vi "imaging_echoes__2743b9f66e.vi"(6 "offset (sec)":dbl=0.005, 7 "trigger voltage":dbl=3.8 format="%0.2f", 9 "frames/period":dbl=10.0, 10 "Exposure (s)":dbl=0.0001, 11 "frequency":dbl) -> (3 "output array":cluster{dbl, dbl}[](array[cluster]))   [LabVIEW 2023]
uses:
  <vilib>/Utility/error.llb/DialogType.ctl
  <vilib>/DAQmx/write.llb/DAQmx Write (Analog DBL 1Chan 1Samp).vi
  <vilib>/DAQmx/write.llb/DAQmx Write (Counter 1D Time 1Chan NSamp).vi
  <vilib>/DAQmx/create/channels.llb/DAQmx Create Channel (AO-Voltage-Basic).vi
  <vilib>/DAQmx/miscellaneous.llb/DAQmx Fill In Error Info.vi
  <vilib>/DAQmx/create/channels.llb/DAQmx Create Channel (CO-Pulse Generation-Time).vi
  <vilib>/DAQmx/configure/trigger.llb/DAQmx Start Trigger (Digital Edge).vi
  <vilib>/DAQmx/configure/timing.llb/DAQmx Timing (Implicit).vi
  <resource>/objmgr/daqmx.rc
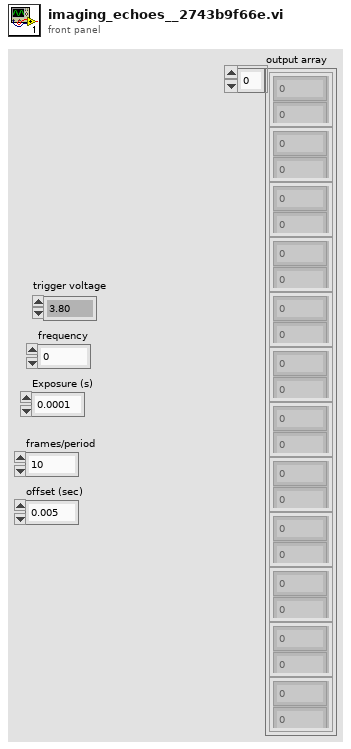
[diagram p1: front panel]
types:
  T1 = typedef "DialogType.ctl" = u16
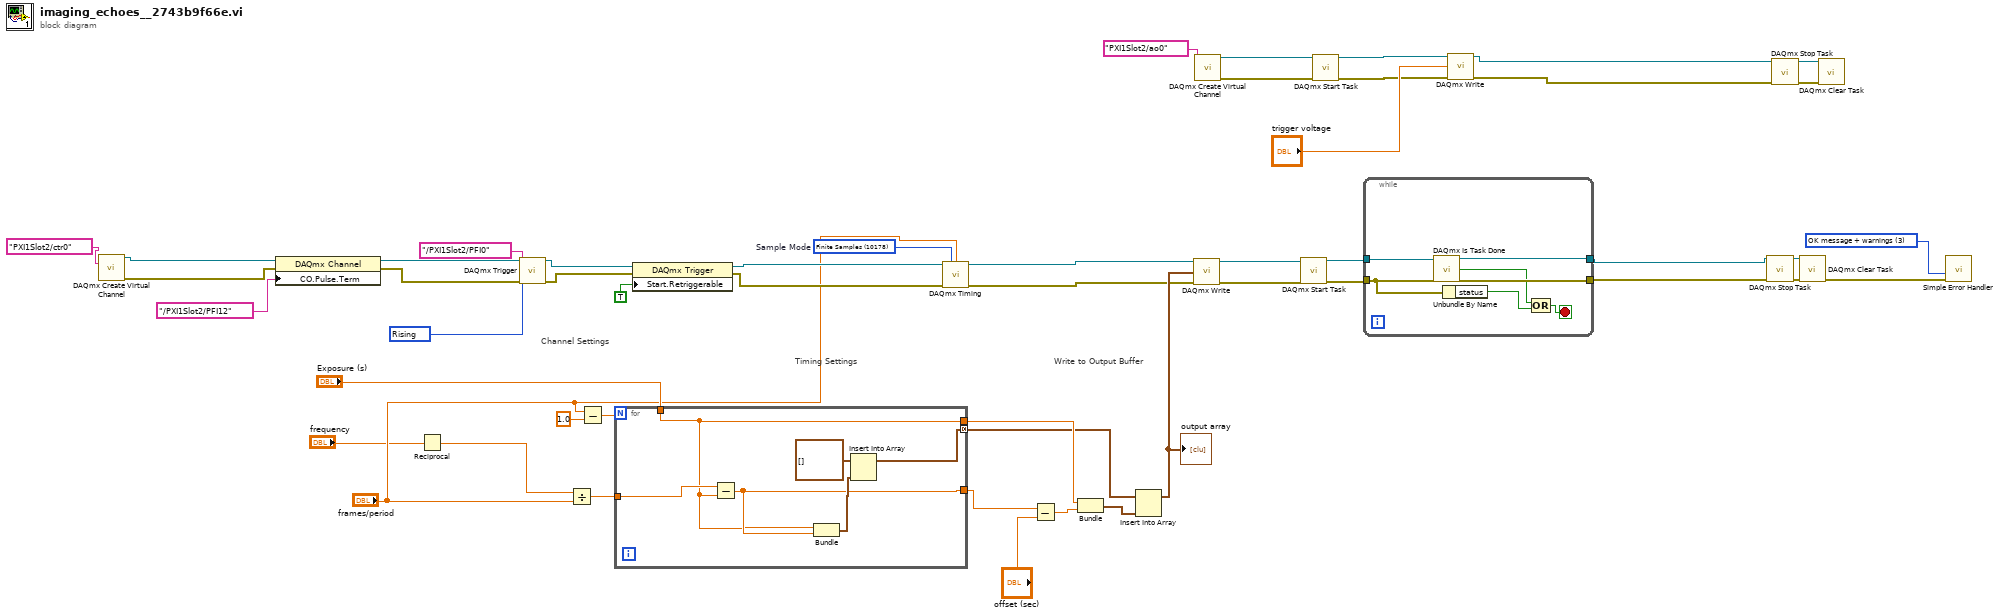
[diagram p0: block diagram]
diagram:
  w47 = 10178 items=["Finite Samples"=10178, "Continuous Samples"=10123, "Hardware Timed Single Point"=12522]  # Sample Mode
  w15 = 10280 items=["Rising"=10280, "Falling"=10171] ("edge")
  w11 = T1 3 items=["no dialog", "OK message", "continue or stop message", "OK message + warnings", "continue/stop + warnings"] ("type of dialog (OK msg:1)")
  # "Write to Output Buffer"
  # "Timing Settings"
  # "Channel Settings"
  n1 = call-poly <vilib>:"DAQmx Create Virtual Channel.vi"("counter"=tag "PXI1Slot2/ctr0") -> ("task out"=w49:refnum<k21>, "error out"=w50:errorcluster)  [unwired: 13 in]
  n2 = property class="DAQmx Channel"(reference=w49, error in=w50, "CO.Pulse.Term"=tag "/PXI1Slot2/PFI12") -> (reference out=w12:refnum<k21>, error out=w13:errorcluster)
  n3 = Reciprocal(x="frequency") -> (1/x=w44:dbl)
  n4 = call-poly <vilib>:"DAQmx Trigger.vi"("task/channels in"=w12, "source"=tag "/PXI1Slot2/PFI0", "edge"=w15, "error in"=w13) -> ("task out"=w16:refnum<k21>, "error out"=w17:errorcluster)  [unwired: 10 in]
  n5 = Divide(x=w44, y="frames/period") -> (x/y=w19:dbl)
  n6 = Subtract(x="frames/period", y=1.0) -> (x-y=w20:dbl)
  n7 = for {
    N: w20 -> [_]
    tunnel: [w54] -> w24 mode=concatenating
    tunnel: w19 -> [w56]
    tunnel: [w52] -> w22
    tunnel: [w51] -> w25
    tunnel: "Exposure (s)" -> [w51]
    n8 = Subtract(x=w56, y=w51) -> (x-y=w52:dbl)
    n9 = Bundle("Exposure (s)"=w51, w52) -> (w55:cluster{"Exposure (s)":dbl, dbl})  [unwired: 1 in]
    n10 = Insert Into Array(array=cluster{dbl, dbl}[] [], new element=w55) -> (w54:cluster{dbl, dbl}[])  [unwired: 1 in]
  }
  n11 = property class="DAQmx Trigger"(reference=w16, error in=w17, "Start.Retriggerable"=TRUE) -> (reference out=w40:refnum<k21>, error out=w41:errorcluster)
  n12 = call-poly <vilib>:"DAQmx Timing.vi"("task/channels in"=w40, "sample mode"=w47, "samples per channel"="frames/period", "error in"=w41) -> ("task out"=w8:refnum<k21>, "error out"=w7:errorcluster)  [unwired: 10 in]
  n13 = Subtract(x=w22, y="offset (sec)") -> (x-y=w23:dbl)
  n14 = Bundle("Exposure (s)"=w25, w23) -> (w26:cluster{"Exposure (s)":dbl, dbl})  [unwired: 1 in]
  n15 = Insert Into Array(array=w24, new element=w26) -> (w27:cluster{dbl, dbl}[])  [unwired: 1 in]
  "output array" <- w27
  n16 = call-poly <vilib>:"DAQmx Write.vi"("task/channels in"=w8, "data"=w27, "error in"=w7) -> ("task out"=w45:refnum<k21>, "error out"=w46:errorcluster)  [unwired: 10 in, 1 out]
  n17 = call-poly <vilib>:"DAQmx Create Virtual Channel.vi"("physical channels"=tag "PXI1Slot2/ao0") -> ("task out"=w31:refnum<k21>, "error out"=w32:errorcluster)  [unwired: 13 in]
  n18 = call <vilib>:"DAQmx Start Task.vi"("task/channels in"=w45, "error in"=w46) -> ("task out"=w4:refnum<k21>, "error out"=w3:errorcluster)  [unwired: 12 in]
  n19 = call <vilib>:"DAQmx Start Task.vi"("task/channels in"=w31, "error in"=w32) -> ("task out"=w33:refnum<k21>, "error out"=w34:errorcluster)  [unwired: 12 in]
  n20 = while {
    tunnel: w4 -> [w61]
    tunnel: w3 -> [w58]
    tunnel: [w59] -> w1
    tunnel: [w60] -> w2
    stop <- w63 stop-if-true
    n21 = call <vilib>:"DAQmx Is Task Done.vi"("task/channels in"=w61, "error in"=w58) -> ("task out"=w60:refnum<k21>, "task done?"=w57:bool, "error out"=w59:errorcluster)  [unwired: 11 in]
    n22 = Unbundle By Name(w58) -> ("status"=w62:bool)
    n23 = Compound Arithmetic op=OR(w57, w62) -> (w63:bool)
  }
  n24 = call-poly <vilib>:"DAQmx Write.vi"("task/channels in"=w33, "data"="trigger voltage", "error in"=w34) -> ("task out"=w35:refnum<k21>, "error out"=w36:errorcluster)  [unwired: 10 in, 1 out]
  n25 = call <vilib>:"DAQmx Stop Task.vi"("task/channels in"=w2, "error in"=w1) -> ("task out"=w9:refnum<k21>, "error out"=w10:errorcluster)  [unwired: 12 in]
  n26 = call <vilib>:"DAQmx Stop Task.vi"("task/channels in"=w35, "error in"=w36) -> ("task out"=w37:refnum<k21>, "error out"=w38:errorcluster)  [unwired: 12 in]
  n27 = call <vilib>:"DAQmx Clear Task.vi"("task in"=w9, "error in"=w10) -> ("error out"=w6:errorcluster)  [unwired: 13 in]
  n28 = call <vilib>:"DAQmx Clear Task.vi"("task in"=w37, "error in"=w38) -> ()  [unwired: 13 in, 1 out]
  n29 = call <vilib>:"Simple Error Handler.vi"("type of dialog (OK msg:1)"=w11, "error in (no error)"=w6) -> ()  [unwired: 3 in, 5 out]
